vi "M1509_DataRead.vi"(1 "Value":u16[][](array[numeric]), 3 "Error In":errorcluster caption="에러 입력(에러 없음)") -> (7 "Robot-M1509 2":T1, 10 "에러 출력":errorcluster)   [LabVIEW 2019]
panel:
  in  "Robot-M1509 3":T1
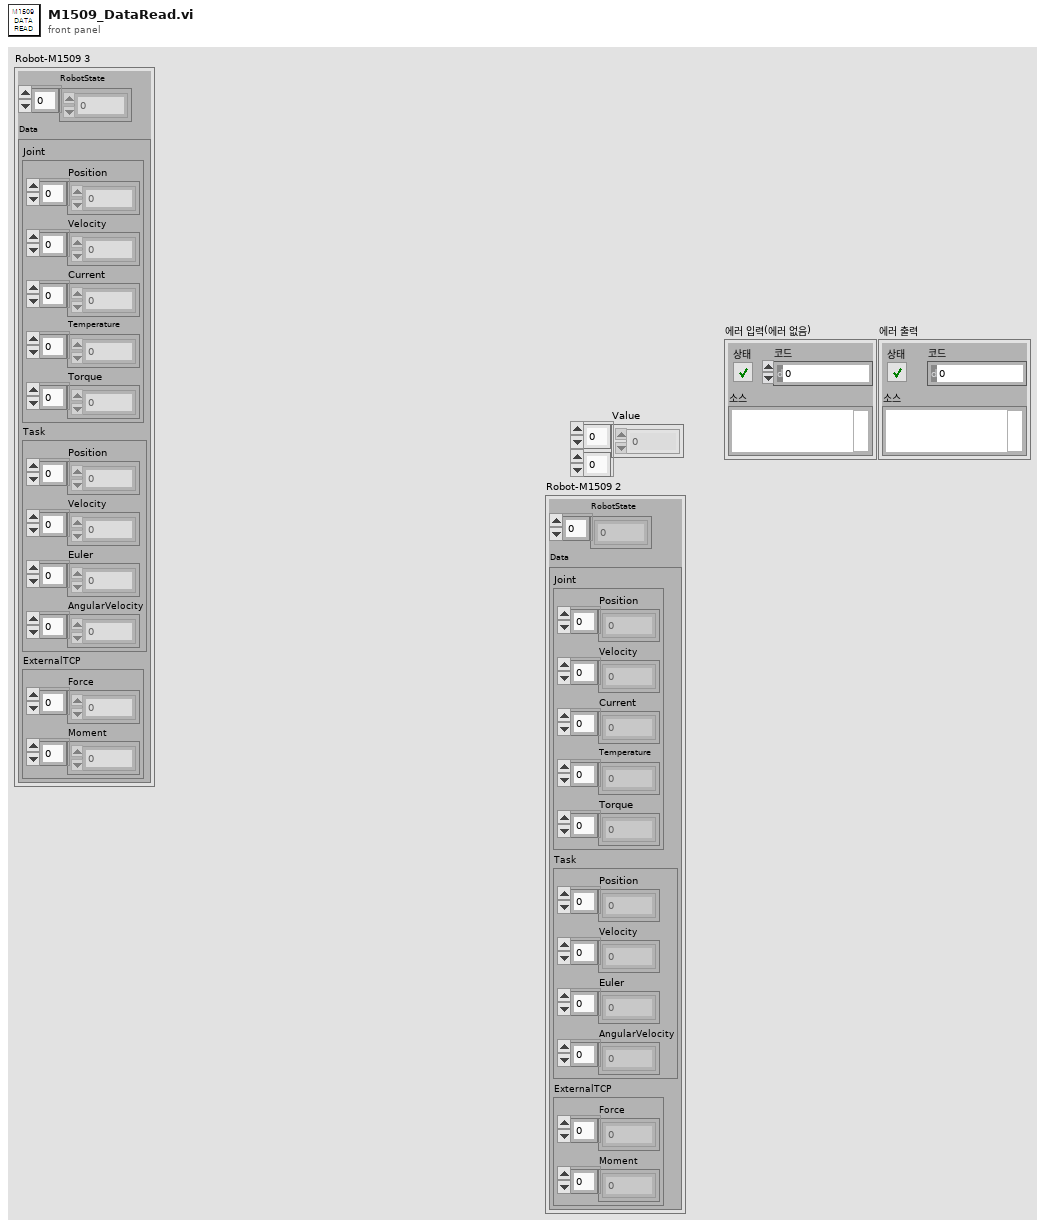
[diagram p1: front panel]
types:
  T1 = cluster{"RobotState":dbl[], "Data":cluster{"Joint":cluster{"Position":dbl[], "Velocity":dbl[], "Current":dbl[], "Temperature":dbl[], "Torque":dbl[]}, "Task":cluster{"Position":dbl[], "Velocity":dbl[], "Euler":dbl[], "AngularVelocity":dbl[]}, "ExternalTCP":cluster{"Force":dbl[], "Moment":dbl[]}}}
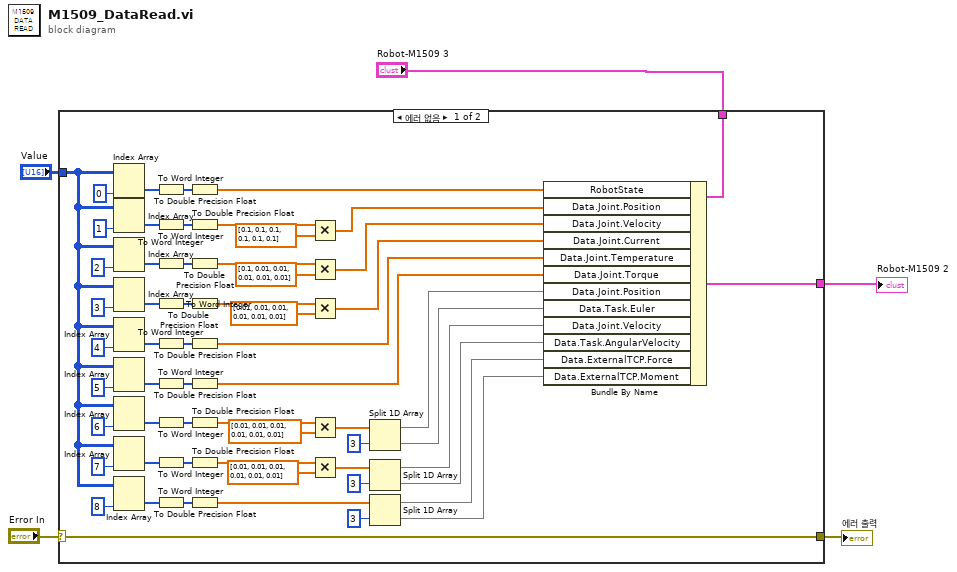
[diagram p0: block diagram]
diagram:
  n1 = case shown="에러 없음" "Error In" {
    selector: "Error In" -> [w8 w65]
    tunnel: [w64 _] -> w1
    tunnel: "Value" -> [w29 _]
    tunnel: [w8 w65] -> w3
    tunnel: "Robot-M1509 3" -> [w6 _]
    frame No Error {
      n2 = Index Array(array=w29, index (col)=0 ("비활성화된 인덱스 (열)")) -> (element=w14:u16[])  [unwired: 1 in]
      n3 = Index Array(array=w29, index (col)=1 ("비활성화된 인덱스 (열)")) -> (element=w11:u16[])  [unwired: 1 in]
      n4 = Index Array(array=w29, index (col)=2 ("비활성화된 인덱스 (열)")) -> (element=w15:u16[])  [unwired: 1 in]
      n5 = Index Array(array=w29, index (col)=3 ("비활성화된 인덱스 (열)")) -> (element=w18:u16[])  [unwired: 1 in]
      n6 = Index Array(array=w29, index (col)=4 ("비활성화된 인덱스 (열)")) -> (element=w19:u16[])  [unwired: 1 in]
      n7 = Index Array(array=w29, index (col)=5 ("비활성화된 인덱스 (열)")) -> (element=w22:u16[])  [unwired: 1 in]
      n8 = Index Array(array=w29, index (col)=6 ("비활성화된 인덱스 (열)")) -> (element=w27:u16[])  [unwired: 1 in]
      n9 = Index Array(array=w29, index (col)=7 ("비활성화된 인덱스 (열)")) -> (element=w26:u16[])  [unwired: 1 in]
      n10 = Index Array(array=w29, index (col)=8 ("비활성화된 인덱스 (열)")) -> (element=w23:u16[])  [unwired: 1 in]
      n11 = To Word Integer(number=w14) -> (16bit integer=w13:i16[])
      n12 = To Word Integer(number=w11) -> (16bit integer=w12:i16[])
      n13 = To Word Integer(number=w15) -> (16bit integer=w16:i16[])
      n14 = To Word Integer(number=w18) -> (16bit integer=w17:i16[])
      n15 = To Word Integer(number=w19) -> (16bit integer=w20:i16[])
      n16 = To Word Integer(number=w22) -> (16bit integer=w21:i16[])
      n17 = To Word Integer(number=w27) -> (16bit integer=w28:i16[])
      n18 = To Word Integer(number=w26) -> (16bit integer=w25:i16[])
      n19 = To Word Integer(number=w23) -> (16bit integer=w24:i16[])
      n20 = To Double Precision Float(number=w13) -> (double precision float=w47:dbl[])
      n21 = To Double Precision Float(number=w12) -> (double precision float=w38:dbl[])
      n22 = To Double Precision Float(number=w16) -> (double precision float=w40:dbl[])
      n23 = To Double Precision Float(number=w17) -> (double precision float=w42:dbl[])
      n24 = To Double Precision Float(number=w20) -> (double precision float=w50:dbl[])
      n25 = To Double Precision Float(number=w21) -> (double precision float=w51:dbl[])
      n26 = To Double Precision Float(number=w28) -> (double precision float=w44:dbl[])
      n27 = To Double Precision Float(number=w25) -> (double precision float=w46:dbl[])
      n28 = To Double Precision Float(number=w24) -> (double precision float=w60:dbl[])
      n29 = Multiply(x=w38, y=dbl[] [0.1, 0.1, 0.1, 0.1, 0.1, 0.1]) -> (x*y=w7:dbl[])
      n30 = Multiply(x=w40, y=dbl[] [0.1, 0.01, 0.01, 0.01, 0.01, 0.01]) -> (x*y=w48:dbl[])
      n31 = Multiply(x=w42, y=dbl[] [0.01, 0.01, 0.01, 0.01, 0.01, 0.01]) -> (x*y=w49:dbl[])
      n32 = Multiply(x=w44, y=dbl[] [0.01, 0.01, 0.01, 0.01, 0.01, 0.01]) -> (x*y=w52:dbl[])
      n33 = Multiply(x=w46, y=dbl[] [0.01, 0.01, 0.01, 0.01, 0.01, 0.01]) -> (x*y=w57:dbl[])
      n34 = Split 1D Array(array=w52, index=3 ("인덱스")) -> (first subarray=w54:dbl[], second subarray=w55:dbl[])
      n35 = Split 1D Array(array=w57, index=3 ("인덱스")) -> (first subarray=w58:dbl[], second subarray=w59:dbl[])
      n36 = Split 1D Array(array=w60, index=3 ("인덱스")) -> (first subarray=w61:dbl[], second subarray=w62:dbl[])
      n37 = Bundle By Name(cluster=w6, "RobotState"=w47, "Data.Joint.Position"=w7, "Data.Joint.Velocity"=w48, "Data.Joint.Current"=w49, "Data.Joint.Temperature"=w50, "Data.Joint.Torque"=w51, "Data.Joint.Position"=w54, "Data.Task.Euler"=w55, "Data.Joint.Velocity"=w58, "Data.Task.AngularVelocity"=w59, "Data.ExternalTCP.Force"=w61, "Data.ExternalTCP.Moment"=w62) -> (w64:T1)
    }
    frame Error {
    }
  }
  "에러 출력" <- w3
  "Robot-M1509 2" <- w1
